vi "Write Event Ref.vi"(8 "error in (no error)":errorcluster, 10 "Event Ref":refnum<user-event>, 11 "UserEventActivationHandler in":refnum<class "UserEventActivationHandler.lvclass">) -> (0 "error out":errorcluster, 3 "UserEventActivationHandler out":refnum<class "UserEventActivationHandler.lvclass">)   [LabVIEW 2026, in "ToastNotification.lvlib" / "UserEventActivationHandler.lvclass"]
uses:
  UserEventActivationHandler.lvclass
  Activation Event Data.ctl
  ToastNotification/Activation.ctl
  ToastNotification/Argument.ctl
  UserEventActivationHandler.lvclass/UserEventActivationHandler.ctl
  ToastNotification/ToastNotification.lvlib
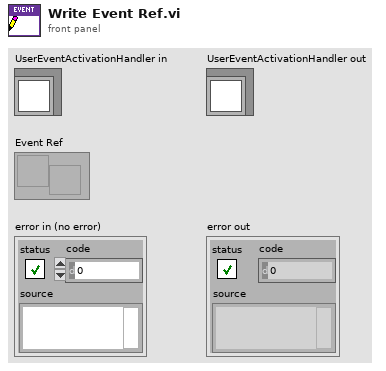
[diagram p1: front panel]
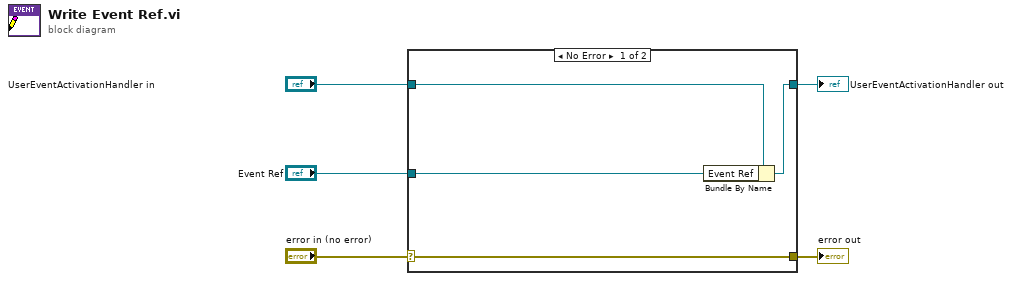
[diagram p0: block diagram]
diagram:
  n1 = case shown="No Error" "error in (no error)" {
    selector: "error in (no error)" -> [w9 w10]
    tunnel: [w9 w10] -> w4
    tunnel: [w7 w11] -> w2
    tunnel: "UserEventActivationHandler in" -> [w8 w11]
    tunnel: "Event Ref" -> [w6 _]
    frame No Error {
      n2 = Bundle By Name(cluster=w8, "Event Ref"=w6) -> (w7:refnum<class "UserEventActivationHandler.lvclass">)
    }
    frame Error {
    }
  }
  "error out" <- w4
  "UserEventActivationHandler out" <- w2
